vi "UE_Can_Advance_Step.vi"(8 "no_fault":bool, 9 "stabilized":bool, 10 "feedback_condition":bool, 11 "quality_valid":bool) -> (3 "advance":bool)   [LabVIEW 2026]
doc: "INTENT: Combine signal quality, required feedback, stabilization and no-fault gate. INPUTS: quality_valid (bool), feedback_condition (bool), stabilized (bool), no_fault (bool). OUTPUTS: advance (bool). DESIGN CONSTRAINT: Sequence scheduler supplies timestamp and timeouts independently. REQUIREMENTS: SRS-F-005, SRS-F-022. No physical hardware side effects. Acceptance requires native LabVIEW compilation and behavioral testing."
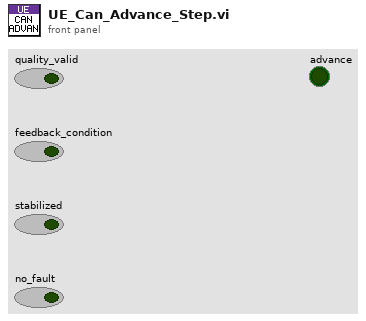
[diagram p1: front panel]
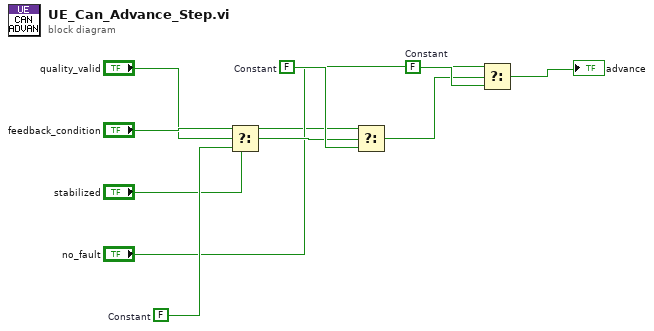
[diagram p0: block diagram]
diagram:
  w9 = FALSE  # Constant
  w7 = FALSE  # Constant
  w5 = FALSE  # Constant
  n1 = Select(t="feedback_condition", s="quality_valid", f=w5) -> (s? t:f=w6:bool)
  n2 = Select(t="stabilized", s=w6, f=w7) -> (s? t:f=w8:bool)
  n3 = Select(t="no_fault", s=w8, f=w9) -> (s? t:f=→"advance":bool)
